vi "I2C Message Buffer - Dequeue.vi"(8 "error in (no error)":errorcluster) -> (0 "error out":errorcluster, 3 "I2C Transaction":string[][](array[string]))   [LabVIEW 2025, in "I2C Bus Monitor.lvclass"]
uses:
  I2C Bus Monitor.lvclass
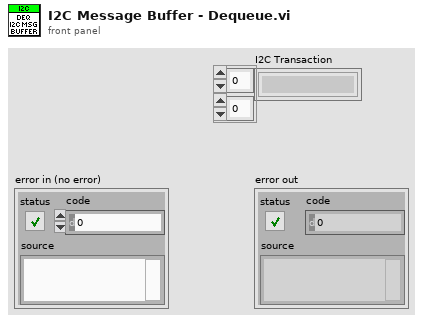
[diagram p1: front panel]
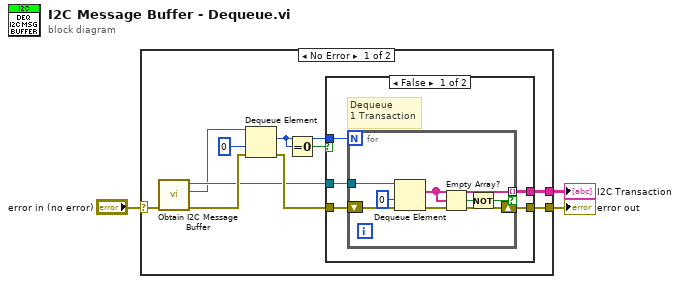
[diagram p0: block diagram]
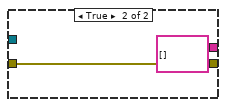
[diagram p2: hidden frame]
diagram:
  n1 = case shown="No Error" "error in (no error)" {
    selector: "error in (no error)" -> [w7 w28]
    tunnel: [w13 w28] -> w3
    tunnel: [w11 _] -> w2
    frame No Error {
      n2 = call "Obtain I2C Message Buffer.vi"("error in (no error)"=w7) -> ("error out"=w6:errorcluster, "Msgs per Txn Queue"=w4:refnum<queue>, "I2C Message Queue"=w5:refnum<queue>)  [unwired: 8 in]
      n3 = Dequeue Element(queue=w4, timeout in ms (-1)=0, error in (no error)=w6) -> (element=w8:i32, error out=w12:errorcluster)  [unwired: 2 out]
      n4 = Equal To 0?(x=w8) -> (x = 0?=w9:bool)
      n5 = case shown="False" w9 {
        tunnel: [w18 w27] -> w13
        tunnel: w12 -> [w17 w27]
        tunnel: w5 -> [w16 _]
        tunnel: w8 -> [w14 _]
        tunnel: [w15 string[][] [] ("I2C Messages")] -> w11
        frame False {
          # "Dequeue\n1 Transaction"
          n6 = for {
            N: w14 -> [_]
            tunnel: w16 -> [w23]
            shift-right: [w25] -> w18
            shift-left: w17 -> [w24]
            tunnel: [w21] -> w15 mode=indexing if=w19
            n7 = Dequeue Element(queue=w23, timeout in ms (-1)=0, error in (no error)=w24) -> (element=w21:string[], error out=w25:errorcluster)  [unwired: 2 out]
            n8 = Empty Array?(array=w21) -> (empty?=w20:bool)
            n9 = Not(x=w20) -> (.not. x?=w19:bool)
          }
        }
        frame True {
        }
      }
    }
    frame Error {
    }
  }
  "error out" <- w3
  "I2C Transaction" <- w2
